vi "GpuMat Upload_HostMem.vi"(8 "error in (no error)":errorcluster, 9 "Stream in":refnum<class "Stream.lvclass">, 10 "HostMem":refnum<class "HostMem.lvclass">, 11 "GpuMat in":refnum<class "GpuMat.lvclass">) -> (0 "error out":errorcluster, 1 "Stream out":refnum<class "Stream.lvclass">, 3 "GpuMat out":refnum<class "GpuMat.lvclass">)   [LabVIEW 2020, in "OpenLvVision_OpenCv.lvlib" / "Cuda.lvlib" / "GpuMat.lvclass"]
doc: "Transfers data from a page-locked (pinned) host memory buffer (HostMem) to the GPU device memory (GpuMat). Using pinned memory is highly recommended for data transfers as it allows for much faster bandwidth. If a valid Stream reference is provided, the upload will execute asynchronously, allowing the CPU to continue working while the transfer occurs."
uses:
  GpuMat.lvclass
  C:/Users/lukas/Documents/OpenLvVision_OpenCv/SourceCode/LabView/OpenLvVision_OpenCv/_LvHelpers/EdvrObject/EdvrObject.lvclass
  HostMem/HostMem.lvclass
  Stream/Stream.lvclass
  _LvHelpers/EdvrObject/EdvrObject.lvclass/EdvrObject.ctl
  OpenLvVision_OpenCv.lvlib
  <vilib>/Utility/error.llb/Error Cluster From Error Code.vi
  <vilib>/ErrorRing/Error Ring.xnode
  _LvHelpers/EdvrObject/EdvrObject.lvclass
  Dlls/OlvOpenCvWrapper.dll
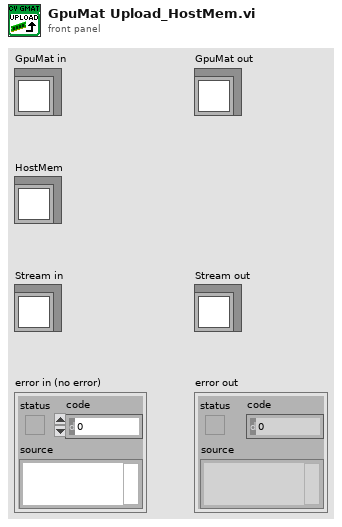
[diagram p1: front panel]
types:
  T1 = typedef "OpenLvVision_OpenCv.lvlib/EdvrObject.lvclass/Edvr.ctl" = refnum<data-value>
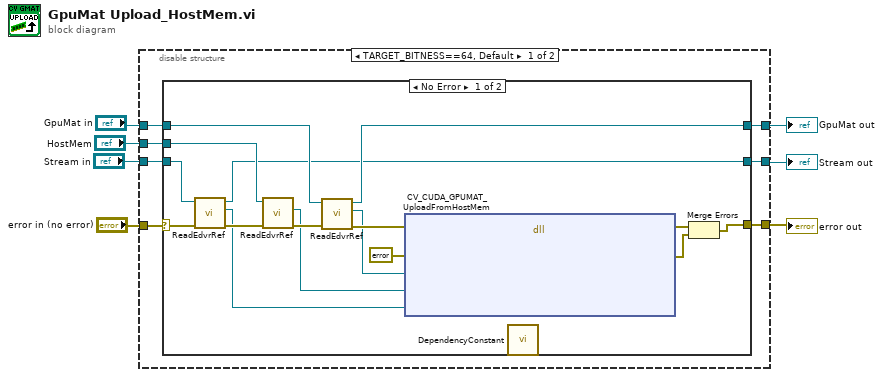
[diagram p0: block diagram]
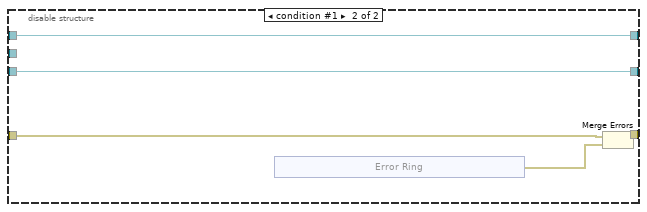
[diagram p3: hidden frame]
diagram:
  n1 = disable-structure shown="TARGET_BITNESS==64, Default" {
    disable-tunnel: "error in (no error)" -> [w14 w37]
    disable-tunnel: [w13 w38] -> w7
    disable-tunnel: "GpuMat in" -> [w12 w34]
    disable-tunnel: [w11 w34] -> w4
    disable-tunnel: "HostMem" -> [w10 _]
    disable-tunnel: "Stream in" -> [w9 w35]
    disable-tunnel: [w8 w35] -> w1
    frame condition #0 (active) {
      n2 = case shown="No Error" w14 {
        selector: w14 -> [w22 w33]
        tunnel: [w27 w33] -> w13
        tunnel: w12 -> [w25 w31]
        tunnel: [w23 w31] -> w11
        tunnel: w10 -> [w19 _]
        tunnel: w9 -> [w18 w32]
        tunnel: [w15 w32] -> w8
        frame No Error {
          n3 = call "ReadEdvrRef.vi"("error in (no error)"=w22, "EdvrObject in"=w18) -> ("error out"=w21:errorcluster, "Edvr"=w16:T1, "EdvrObject out"=w15:refnum<class "Stream.lvclass">)  [unwired: 7 in]
          n4 = call "ReadEdvrRef.vi"("error in (no error)"=w21, "EdvrObject in"=w19) -> ("error out"=w20:errorcluster, "Edvr"=w17:T1)  [unwired: 7 in, 1 out]
          n5 = call "ReadEdvrRef.vi"("error in (no error)"=w20, "EdvrObject in"=w25) -> ("error out"=w26:errorcluster, "Edvr"=w24:T1, "EdvrObject out"=w23:refnum<class "GpuMat.lvclass">)  [unwired: 7 in]
          n6 = dll-call lib="C:/Users/lukas/Documents/OpenLvVision_OpenCv/SourceCode/LabView/OpenLvVision_OpenCv/Dlls/OlvOpenCvWrapper.dll" fn="CV_CUDA_GPUMAT_UploadFromHostMem"(error in=w26, "Error"=errorcluster {"status"=FALSE, "code"=0, "source"=""} ("error out"), "edvrRef"=w24, "hostMemRef"=w17, "streamRef"=w16) -> (error out=w30:errorcluster, "Error"=w29:errorcluster)  [unwired: 6 in, 1 out]
          n7 = call "DependencyConstant.vi"() -> ()  [unwired: 12 in]
          n8 = Merge Errors(w30, w29) -> (w27:errorcluster)
        }
        frame Error {
        }
      }
    }
    frame condition #1 {
      n9 = xnode "Error Ring"() -> ("error out"=w36:errorcluster)
      n10 = Merge Errors(w37, w36) -> (w38:errorcluster)
    }
  }
  "error out" <- w7
  "GpuMat out" <- w4
  "Stream out" <- w1
